vi "etl-mpc_matlab.vi"(2 "AO Sample Period":dbl=1e-06, 4 "model file path":path=path "C:/WormSPIM/Labview/SPIM Engine/Scan generators/etl_model_v1.0.mat", 5 "volume period":dbl, 6 "frame period":dbl=0.006, 7 "slice array":dbl[](array[numeric])) -> (0 "Predicted Scan Path":dbl[](array[numeric]), 1 "ETL scan waveform":dbl[](array[numeric]))   [LabVIEW 2020, in "Scan Generators.lvlib"]
uses:
  Scan Generators.lvlib
panel:
  out "Waveform Graph 2":waveform(dbl)(graph)
  out "Waveform Graph":waveform(dbl)(graph)
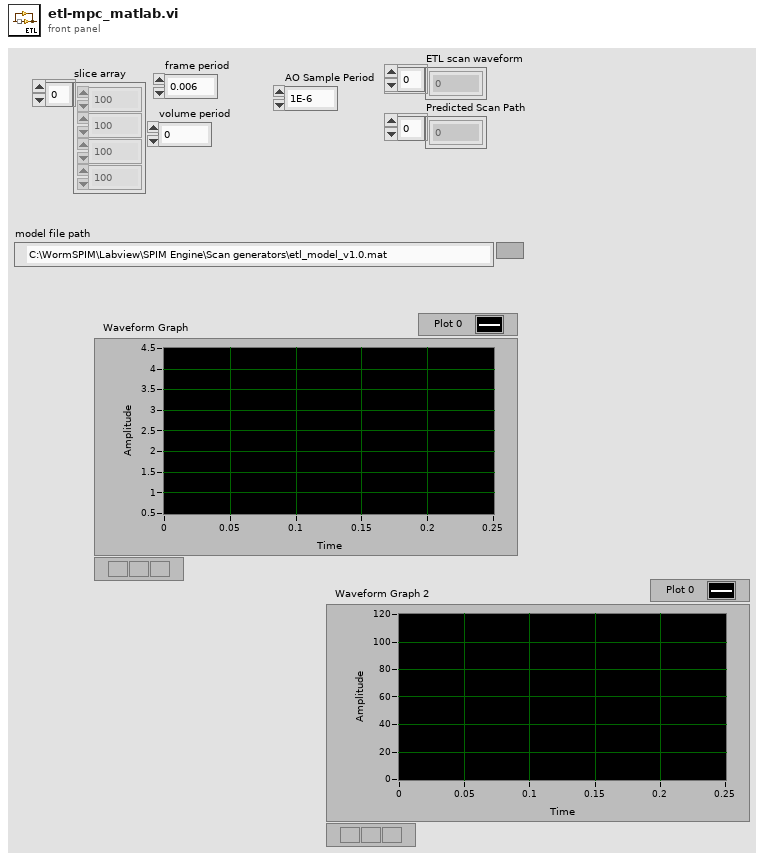
[diagram p1: front panel]
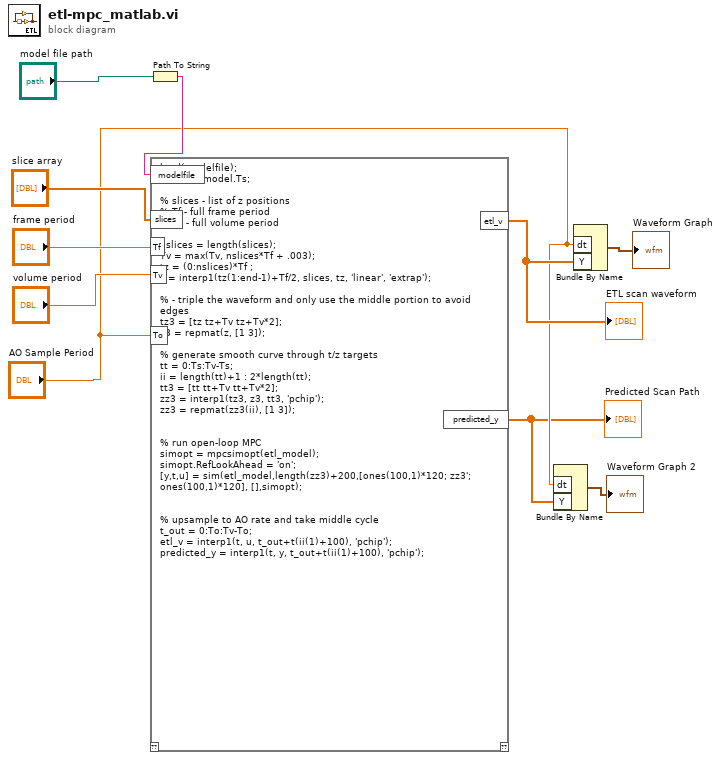
[diagram p0: block diagram]
diagram:
  n1 = Path To String(path="model file path") -> (string=w7:string)
  n2 = script code="load(modelfile);\nTs = etl_model.Ts;\n\n% slices - list of z positions\n% Tf - full frame period\n% Tv - full volume period\n\nnslices = length(slices);\nTv = max(Tv, nslices*Tf + .003);\ntz = (0:nslices)*Tf ;\nz = interp1(tz(1:end-1)+Tf/2, slices, tz, 'linear', 'extrap');\n\n% - triple the waveform and only use the middle portion to avoid edges\ntz3 = [tz tz+Tv tz+Tv*2];\nz3 = repmat(z, [1 3]);\n\n% generate smooth curve through t/z targets\ntt = 0:Ts:Tv-Ts;\nii = length(tt)+1 : 2*length(tt);\ntt3 = [tt tt+Tv tt+Tv*2];\nzz3 = interp1(tz3, z3, tt3, 'pchip');\nzz3 = repmat(zz3(ii), [1 3]);\n\n\n% run open-loop MPC\nsimopt = mpcsimopt(etl_model);\nsimopt.RefLookAhead = 'on';\n[y,t,u] = sim(etl_model,length(zz3)+200,[ones(100,1)*120; zz3'; ones(100,1)*120], [],simopt);\n\n\n% upsample to AO rate and take middle cycle\nt_out = 0:To:Tv-To;\netl_v = interp1(t, u, t_out+t(ii(1)+100), 'pchip');\npredicted_y = interp1(t, y, t_out+t(ii(1)+100), 'pchip');"("slices"="slice array", "Tf"="frame period", "Tv"="volume period", "modelfile"=w7, "To"="AO Sample Period") -> ("etl_v"=w6:dbl[], "predicted_y"=w2:dbl[])  [unwired: 1 in, 1 out]
  "ETL scan waveform" <- w6
  "Predicted Scan Path" <- w2
  n3 = Bundle By Name("dt"="AO Sample Period", "Y"=w2) -> (→"Waveform Graph 2":waveform(dbl))  [unwired: 1 in]
  n4 = Bundle By Name("dt"="AO Sample Period", "Y"=w6) -> (→"Waveform Graph":waveform(dbl))  [unwired: 1 in]
